vi "test internal error message.vi"(8 "error in (no error)":errorcluster) -> (0 "error out":errorcluster, 3 "body":string)   [LabVIEW 2020, in "MCP Server tests.lvlib"]
doc: "The message of an internal error (-32603) must not contain a VI call chain (->), <b> markup, <APPEND> or <ERR> tags or a file path. Checked with a prompt whose VI is not executable."
uses:
  MCP Server tests.lvlib
  8769857c-2ecc-4015-a67f-a4a613aa06ca.vi
  <vilib>/JDP Science/JSONtext/Next JSON Value.vi
  <vilib>/JDP Science/JSONtext/String Subset.vi
  <vilib>/JDP Science/JSONtext/Parsing/Advance past next JSON Value (inlined COPY).vi
  <vilib>/JDP Science/JSONtext/Parsing/Advance past whitespace.vi
  <vilib>/JDP Science/JSONtext/Parsing/Advance past String.vi
  <vilib>/JDP Science/JSONtext/Parsing/Advance past Number.vi
  <vilib>/JDP Science/JSONtext/Parsing/Advance past Line Ending.vi
  <vilib>/JDP Science/JSONtext/Parsing/Parse Full Path or Item Name.vi
  <vilib>/JDP Science/JSONtext/Parsing/Advance past Array.vi
  <vilib>/JDP Science/JSONtext/Parsing/Advance past Object.vi
  <vilib>/JDP Science/JSONtext/support/Error Cluster From Code.vi
  <vilib>/JDP Science/JSONtext/Offset/Find Item Locations by Path.vi
  <vilib>/JDP Science/JSONtext/JSON text to Variant.vi
  <vilib>/JDP Science/JSONtext/LVClass Serializer/JSONtext LVClass Serializer.lvclass
  <vilib>/addons/_JKI Toolkits/Caraya/classes/Test/Test.lvclass
  <vilib>/JDP Science/JSONtext/JSONtext.lvlib
  <vilib>/addons/_JKI Toolkits/Caraya/classes/Assert/Assert.lvclass
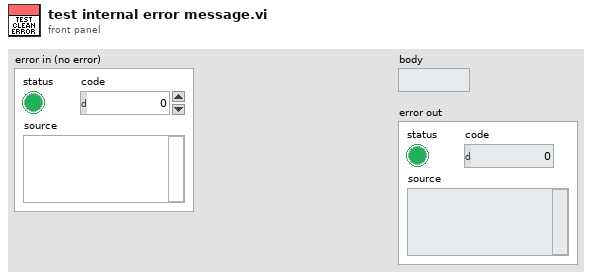
[diagram p1: front panel]
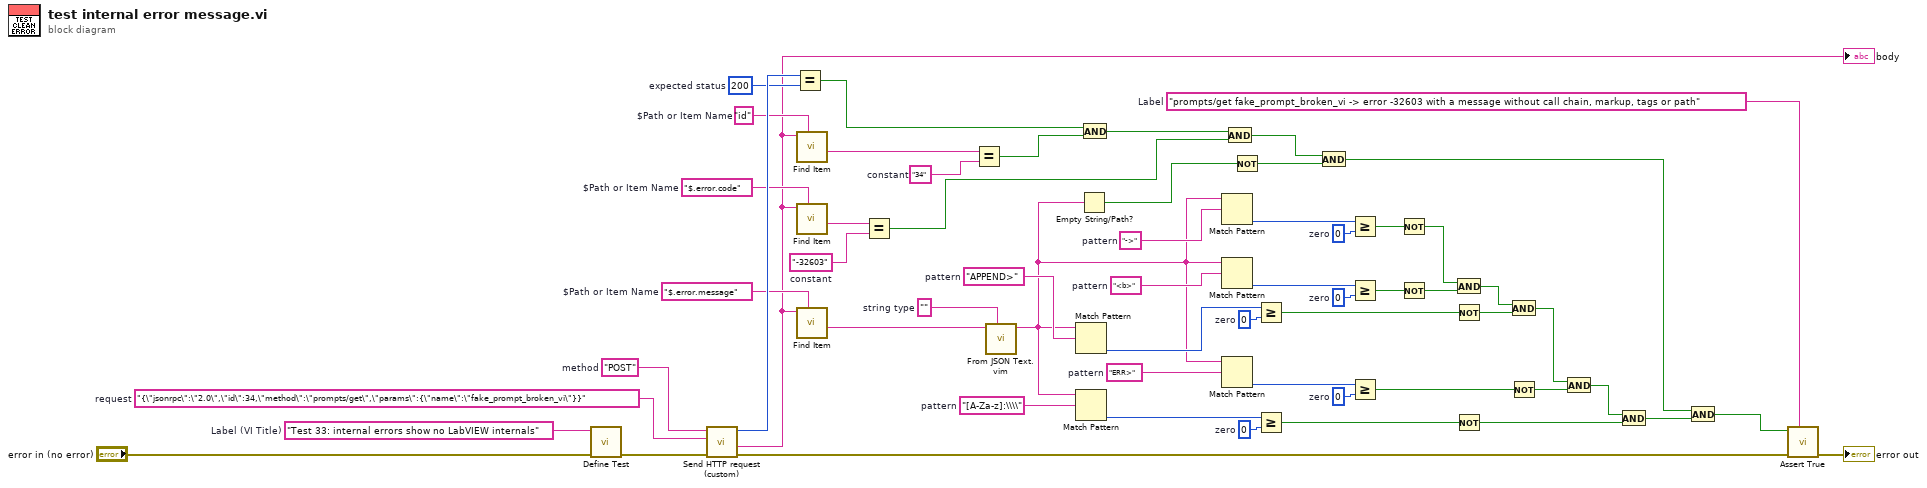
[diagram p0: block diagram]
diagram:
  w3 = "prompts/get fake_prompt_broken_vi -> error -32603 with a message without call chain, markup, tags or path"  # Label
  w16 = "-32603"  # constant
  w18 = "34"  # constant
  w29 = 0  # zero
  w31 = "[A-Za-z]:\\\\"  # pattern
  w33 = 0  # zero
  w35 = "ERR>"  # pattern
  w37 = 0  # zero
  w39 = "APPEND>"  # pattern
  w41 = 0  # zero
  w43 = "<b>"  # pattern
  w45 = 0  # zero
  w47 = "->"  # pattern
  w48 = ""  # string type
  w50 = "$.error.message"  # $Path or Item Name
  w51 = "$.error.code"  # $Path or Item Name
  w52 = "id"  # $Path or Item Name
  w53 = 200  # expected status
  w56 = "{\"jsonrpc\":\"2.0\",\"id\":34,\"method\":\"prompts/get\",\"params\":{\"name\":\"fake_prompt_broken_vi\"}}"  # request
  w57 = "POST"  # method
  w59 = "Test 33: internal errors show no LabVIEW internals"  # Label (VI Title)
  n1 = call <vilib>:"Define Test.vi"("error in (no error)"="error in (no error)", "Label (VI Title)"=w59) -> ("error out"=w55:errorcluster)  [unwired: 8 in, 1 out]
  n2 = call "Send HTTP request (custom).vi"("error in (no error)"=w55, "request"=w56, "method"=w57) -> ("error out"=w4:errorcluster, "response"=w2:string, "status code"=w54:i32)  [unwired: 5 in, 1 out]
  "body" <- w2
  n3 = Equal?(x=w54, y=w53) -> (x = y?=w13:bool)
  n4 = call <vilib>:"Find Item.vi"("$Path or Item Name"=w52, "JSON"=w2) -> ("<JSON>"=w19:string)  [unwired: 6 in, 3 out]
  n5 = call <vilib>:"Find Item.vi"("$Path or Item Name"=w51, "JSON"=w2) -> ("<JSON>"=w17:string)  [unwired: 6 in, 3 out]
  n6 = call <vilib>:"Find Item.vi"("$Path or Item Name"=w50, "JSON"=w2) -> ("<JSON>"=w49:string)  [unwired: 6 in, 3 out]
  n7 = Equal?(x=w17, y=w16) -> (x = y?=w10:bool)
  n8 = Equal?(x=w19, y=w18) -> (x = y?=w12:bool)
  n9 = call "From JSON Text.vim"("Data Type and Default Value"=w48, "JSON"=w49) -> ("Data out"=w15:string)  [unwired: 8 in, 1 out]
  n10 = Match Pattern(string=w15, regular expression=w39) -> (offset past match=w38:i32)  [unwired: 1 in, 3 out]
  n11 = Match Pattern(string=w15, regular expression=w31) -> (offset past match=w30:i32)  [unwired: 1 in, 3 out]
  n12 = Empty String/Path?(string/path=w15) -> (empty?=w14:bool)
  n13 = And(x=w13, y=w12) -> (x .and. y?=w11:bool)
  n14 = Match Pattern(string=w15, regular expression=w47) -> (offset past match=w46:i32)  [unwired: 1 in, 3 out]
  n15 = Match Pattern(string=w15, regular expression=w43) -> (offset past match=w42:i32)  [unwired: 1 in, 3 out]
  n16 = Match Pattern(string=w15, regular expression=w35) -> (offset past match=w34:i32)  [unwired: 1 in, 3 out]
  n17 = And(x=w11, y=w10) -> (x .and. y?=w9:bool)
  n18 = Not(x=w14) -> (.not. x?=w8:bool)
  n19 = Greater Or Equal?(x=w38, y=w37) -> (x >= y?=w36:bool)
  n20 = Greater Or Equal?(x=w30, y=w29) -> (x >= y?=w28:bool)
  n21 = And(x=w9, y=w8) -> (x .and. y?=w7:bool)
  n22 = Greater Or Equal?(x=w46, y=w45) -> (x >= y?=w44:bool)
  n23 = Greater Or Equal?(x=w42, y=w41) -> (x >= y?=w40:bool)
  n24 = Greater Or Equal?(x=w34, y=w33) -> (x >= y?=w32:bool)
  n25 = Not(x=w44) -> (.not. x?=w27:bool)
  n26 = Not(x=w40) -> (.not. x?=w26:bool)
  n27 = And(x=w27, y=w26) -> (x .and. y?=w25:bool)
  n28 = Not(x=w36) -> (.not. x?=w24:bool)
  n29 = Not(x=w28) -> (.not. x?=w20:bool)
  n30 = And(x=w25, y=w24) -> (x .and. y?=w23:bool)
  n31 = Not(x=w32) -> (.not. x?=w22:bool)
  n32 = And(x=w23, y=w22) -> (x .and. y?=w21:bool)
  n33 = And(x=w21, y=w20) -> (x .and. y?=w6:bool)
  n34 = And(x=w7, y=w6) -> (x .and. y?=w5:bool)
  n35 = call <vilib>:"Assert True.vi"("Label"=w3, "error in (no error)"=w4, "True?"=w5) -> ("error out"=→"error out":errorcluster)  [unwired: 7 in, 1 out]
